vi "Get Target ref.vi"(8 "error in (no error)":errorcluster, 10 "Target Name":string, 11 "Project in":refnum<vi>) -> (0 "error out":errorcluster, 2 "Target ref out":refnum<vi>, 3 "Project out":refnum<vi>)   [LabVIEW 2019, in "gRPC Template Creation Utility.lvlib"]
uses:
  gRPC Template Creation Utility.lvlib
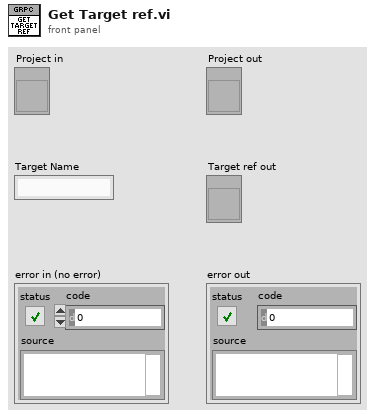
[diagram p1: front panel]
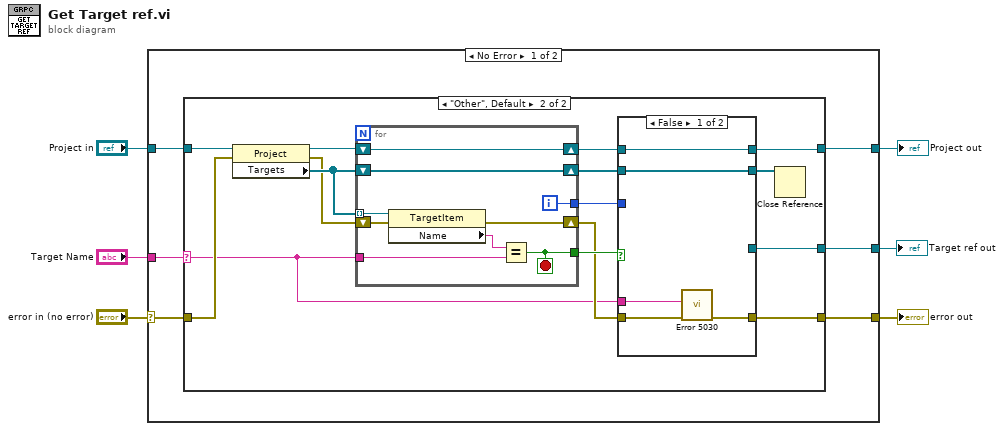
[diagram p0: block diagram]
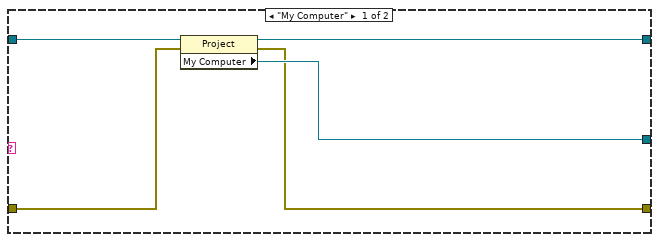
[diagram p2: hidden frame]
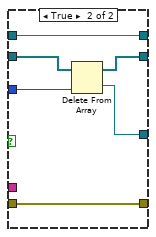
[diagram p3: hidden frame]
diagram:
  n1 = case shown="No Error" "error in (no error)" {
    selector: "error in (no error)" -> [w8 w53]
    tunnel: [w10 w54] -> w6
    tunnel: [w7 w53] -> w5
    tunnel: "Project in" -> [w12 w54]
    tunnel: "Target Name" -> [w11 _]
    tunnel: [w9 _] -> w1
    frame No Error {
      n2 = case shown="\"Other\", Default" w11 {
        selector: w11 -> [_ w20]
        tunnel: w12 -> [w17 w32]
        tunnel: [w16 w18] -> w10
        tunnel: [w15 w22] -> w9
        tunnel: w8 -> [w14 w29]
        tunnel: [w13 w21] -> w7
        frame "My Computer" {
          n3 = property class="Project"(reference=w17, error in=w14) -> (reference out=w16:refnum<vi>, error out=w13:errorcluster, "My Computer"=w15:refnum<vi>)
        }
        frame "Other", Default {
          n4 = property class="Project"(reference=w32, error in=w29) -> (reference out=w31:refnum<vi>, error out=w28:errorcluster, "Targets"=w30:refnum<vi>[])
          n5 = for {
            tunnel: w30 -> [w52] mode=indexing
            shift-right: [w51] -> w19
            shift-left: w31 -> [w51]
            tunnel: w20 -> [w44]
            shift-right: [w48] -> w26
            shift-left: w30 -> [w48]
            shift-right: [w45] -> w24
            shift-left: w28 -> [w49]
            tunnel: [w47] -> w27
            tunnel: [w46] -> w25
            i -> [w46]
            stop <- w47 stop-if-true
            n6 = property class="TargetItem"(reference=w52, error in=w49) -> (error out=w45:errorcluster, "Name"=w50:string)  [unwired: 1 out]
            n7 = Equal?(x=w50, y=w44) -> (x = y?=w47:bool)
          }
          n8 = case shown="False" w27 {
            tunnel: w26 -> [w37 w43]
            tunnel: w25 -> [_ w42]
            tunnel: [w37 w41] -> w23
            tunnel: w24 -> [w36 w39]
            tunnel: [_ w40] -> w22
            tunnel: [w35 w39] -> w21
            tunnel: w20 -> [w34 _]
            tunnel: w19 -> [w33 w38]
            tunnel: [w33 w38] -> w18
            frame False {
              n9 = call "Error 5030.vi"("error in (no error)"=w36, "Target Name"=w34) -> ("error out"=w35:errorcluster)  [unwired: 9 in]
            }
            frame True {
              n10 = Delete From Array(array=w43, index=w42) -> (deleted portion=w40:refnum<vi>, array with subset deleted=w41:refnum<vi>[])  [unwired: 1 in]
            }
          }
          n11 = Close Reference(reference=w23) -> ()  [unwired: 1 in, 1 out]
        }
      }
    }
    frame Error {
    }
  }
  "Project out" <- w6
  "error out" <- w5
  "Target ref out" <- w1
